vi "HELP.vi"(6 "timeout (ms) [500]":i32=500, 8 "error in (no error)":errorcluster, 11 "Instrument in":refnum<class "Instrument.lvclass">) -> (0 "error out":errorcluster, 2 "Commands":string[](array[string]), 3 "Instrument in":refnum<class "Instrument.lvclass">)   [LabVIEW 2019, in "Instrument.lvlib" / "Instrument.lvclass"]
doc: "Send \"HELP\" command to get API supported by remote Instrument."
uses:
  Instrument.lvclass
  Typedefs/Instrument.Commands--Enum.ctl
  dbe59fba-fa6e-4a70-9689-10cf786b7836.vi
  dbe59fba-fa6e-4a70-9689-10cf786b7836.vi/2b178c0d-6d71-4bc5-82bd-bdad18b8f5fd.vi
  dbe59fba-fa6e-4a70-9689-10cf786b7836.vi/e8016165-2873-4a0a-85dd-65ff95e51b5c.vi
  <vilib>/Utility/Data Type/Get Type Information.vi
  <vilib>/JDP Science/JSONtext/JSON text to Variant.vi
  <vilib>/JDP Science/JSONtext/LVClass Serializer/JSONtext LVClass Serializer.lvclass
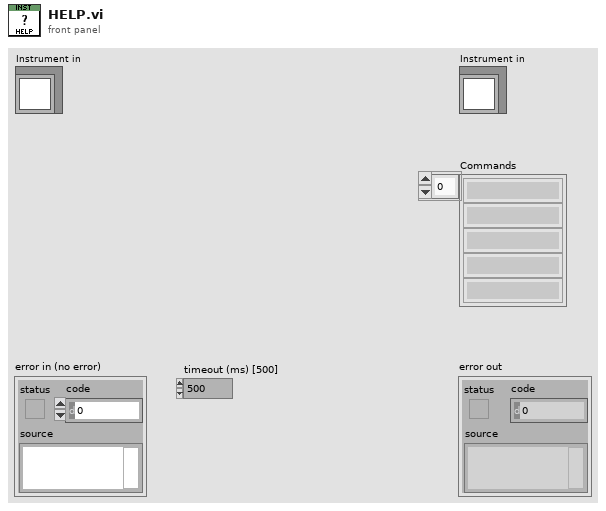
[diagram p1: front panel]
types:
  T1 = typedef "Instrument.lvlib/Instrument.lvclass/Instrument.Commands--Enum.ctl" = enum16{"ACK", "HELP", "IDN", "getAll", "getAllData"}
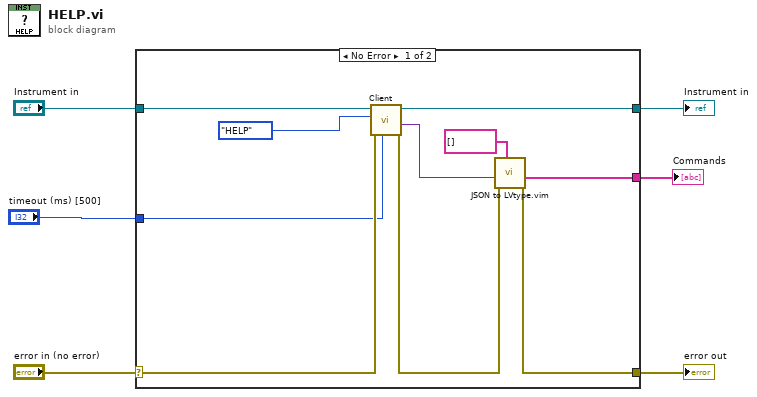
[diagram p0: block diagram]
diagram:
  n1 = case shown="No Error" "error in (no error)" {
    selector: "error in (no error)" -> [w14 w18]
    tunnel: [w10 w18] -> w5
    tunnel: [w16 w17] -> w3
    tunnel: "Instrument in" -> [w15 w17]
    tunnel: [w9 _] -> w2
    tunnel: "timeout (ms) [500]" -> [w7 _]
    frame No Error {
      n2 = call-dynamic "Client.vi"("timeout (ms) [500]"=w7, "error in (no error)"=w14, "Command in"=Instrument.Commands--Enum."HELP" ("Commands"), "Instrument in"=w15) -> ("error out"=w11:errorcluster, "Data out"=w8:variant, "Instrument out"=w16:refnum<class "Instrument.lvclass">)  [unwired: 4 in, 1 out]
      n3 = call "JSON to LVtype.vim"("type"=string[] [] ("Commands"), "error in (no error)"=w11, "JSON Data in"=w8) -> ("error out"=w10:errorcluster, "Data out"=w9:string[])  [unwired: 7 in]
    }
    frame Error {
    }
  }
  "error out" <- w5
  "Instrument in" <- w3
  "Commands" <- w2
